vi "serialization tests.vi"() -> (0 "serialization error":errorcluster, 1 "validation error":errorcluster, 3 "Pass":bool)   [LabVIEW 2015, in "tdms logger tests.lvlib"]
uses:
  tdms logger tests.lvlib
  configuration/TDMS datalogger configuration.lvclass
  configuration/TDMS datalogger configuration.lvclass/TDMS datalogger configuration.ctl
  configuration/Read channels.vi
  <vilib>/NI/Tag Bus Module Framework/channel/TBM channel.lvclass
panel:
  out "lines equal":bool
  out "channels equal":bool
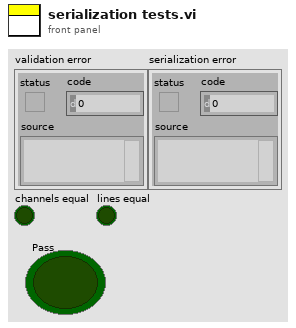
[diagram p1: front panel]
types:
  T1 = cluster{"channel":refnum<class "TBM channel.lvclass">}[]
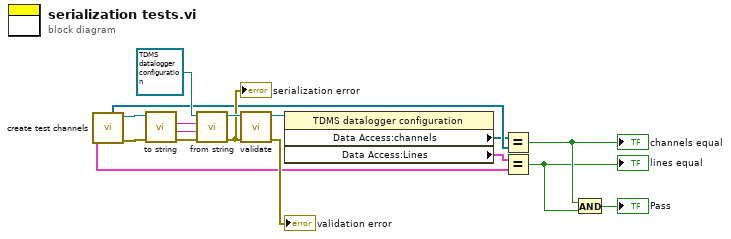
[diagram p0: block diagram]
diagram:
  n1 = call "create test channels.vi"() -> ("error out"=w8:errorcluster, "TDMS datalogger configuration out"=w9:refnum<class "TDMS datalogger configuration.lvclass">, "chans"=w7:refnum<class "TBM channel.lvclass">[], "Lines"=w4:T1)  [unwired: 3 in, 5 out]
  n2 = call-dynamic "to string.vi"("error in"=w8, "TDMS datalogger configuration in"=w9) -> ("error out"=w17:errorcluster, "data"=w16:string, "version"=w15:string)  [unwired: 6 in, 1 out]
  n3 = call-dynamic "from string.vi"("error in"=w17, "data"=w16, "version"=w15, "TDMS datalogger configuration in"=refnum<class "TDMS datalogger configuration.lvclass"> refnum ("TDMS datalogger configuration")) -> ("error out"=w12:errorcluster, "TDMS datalogger configuration out"=w14:refnum<class "TDMS datalogger configuration.lvclass">)  [unwired: 6 in]
  "serialization error" <- w12
  n4 = call-dynamic "validate.vi"("error in"=w12, "TDMS datalogger configuration in"=w14) -> ("error out"=→"validation error":errorcluster, "TDMS datalogger configuration out"=w11:refnum<class "TDMS datalogger configuration.lvclass">)  [unwired: 8 in]
  n5 = property class="TDMS datalogger configuration"(reference=w11) -> ("Data Access:channels"=w6:refnum<class "TBM channel.lvclass">[], "Data Access:Lines"=w5:T1)  [unwired: 1 in, 2 out]
  n6 = Equal?(x=w6, y=w7) -> (x = y?=w3:bool)
  "channels equal" <- w3
  n7 = Equal?(x=w5, y=w4) -> (x = y?=w2:bool)
  "lines equal" <- w2
  n8 = And(x=w3, y=w2) -> (x .and. y?=→"Pass":bool)
